vi "W14_FailRate_test.vi"() -> ()   [LabVIEW 2026]
doc: "Use this template to build a VI to use as a subVI."
panel:
  out "notify (each board)":bool[](array[boolean])
  out "boards in window (each board)":i32[](array[numeric])
  out "FAIL rate % (each board)":dbl[](array[numeric])
  in  "FAIL sequence":bool[](array[boolean])
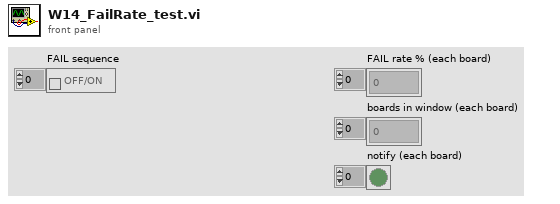
[diagram p1: front panel]
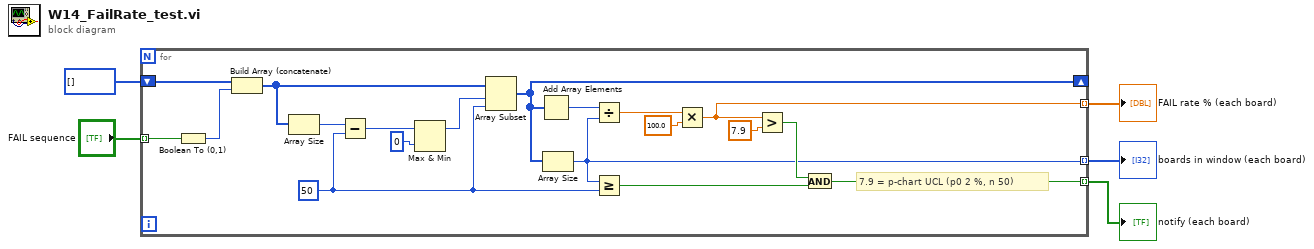
[diagram p0: block diagram]
diagram:
  n1 = for {
    shift-right: [w15] -> _
    shift-left: i16[] [] -> [w23]
    tunnel: "FAIL sequence" -> [w24] mode=indexing
    tunnel: [w8] -> w3 mode=indexing
    tunnel: [w7] -> w2 mode=indexing
    tunnel: [w6] -> w1 mode=indexing
    w19 = 50 ("y")
    # "7.9 = p-chart UCL (p0 2 %, n 50)"
    n2 = Boolean To (0,1)(Boolean=w24) -> (0, 1=w22:i16)
    n3 = Build Array (concatenate)(w23, w22) -> (w21:i16[])
    n4 = Array Size(array=w21) -> (size(s)=w20:i32)
    n5 = Subtract(x=w20, y=w19) -> (x-y=w18:i32)
    n6 = Max & Min(x=w18, y=0) -> (max(x,y)=w16:i32)  [unwired: 1 out]
    n7 = Array Subset(array=w21, index=w16, length=w19) -> (w15:i16[])
    n8 = Add Array Elements(numeric array=w15) -> (sum=w14:i16)
    n9 = Array Size(array=w15) -> (size(s)=w7:i32)
    n10 = Divide(x=w14, y=w7) -> (x/y=w13:dbl)
    n11 = Greater Or Equal?(x=w7, y=w19) -> (x >= y?=w9:bool)
    n12 = Multiply(x=w13, y=100.0) -> (x*y=w8:dbl)
    n13 = Greater?(x=w8, y=7.9) -> (0:w10:bool)
    n14 = And(x=w10, y=w9) -> (x .and. y?=w6:bool)
  }
  "FAIL rate % (each board)" <- w3
  "boards in window (each board)" <- w2
  "notify (each board)" <- w1
